vi "Reinitialize VI Inputs.vi"(8 "error in":errorcluster, 11 "VI in":refnum<vi>) -> (0 "error out":errorcluster, 3 "VI out":refnum<vi>)   [LabVIEW 2020, in "MCP Server.lvlib"]
doc: "Sets every control of a tool or prompt VI back to its default value before the VI is called.\n\nCall VI.vi sets only the inputs that a request gives. Without this step an input that the request leaves out would keep the value of the previous call instead of its default.\n\nAn error of the reset (for example because the VI is running) is not reported here: calling the VI reports it."
uses:
  MCP Server.lvlib
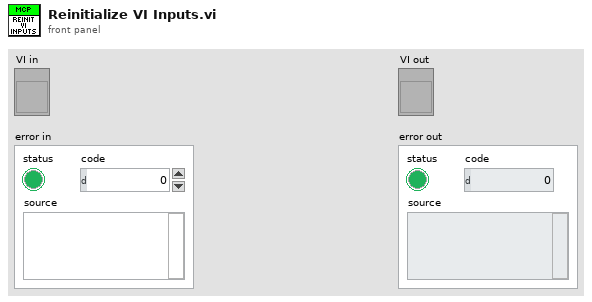
[diagram p1: front panel]
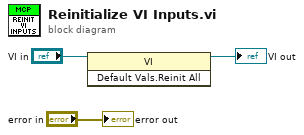
[diagram p0: block diagram]
diagram:
  n1 = invoke class="VI" method="Default Vals.Reinit All"(reference="VI in") -> (reference out=→"VI out":refnum<vi>)  [unwired: 2 in, 2 out]
  "error out" <- "error in"
